vi "Plugin_Validate_Manifest.vi"(8 "error in (no error)":errorcluster={"status"=FALSE, "code"=0, "source"="\"\""}, 10 "target capability":string, 11 "PluginManifest":string) -> (0 "error out":errorcluster={"status"=FALSE, "code"=0, "source"="\"\""}, 2 "status ok":bool, 3 "Allowed/diagnostics":string)   [LabVIEW 2026]
doc: "INTENT: Check plugin interface rights. LOGIC: Check connector signature/version, input/output type, target presence, resource rights and cancellation deadlines."
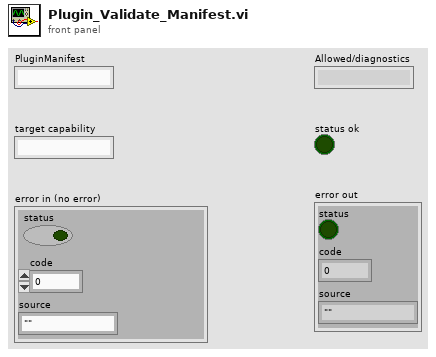
[diagram p1: front panel]
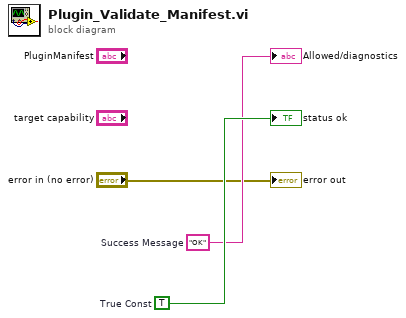
[diagram p0: block diagram]
diagram:
  w3 = TRUE  # True Const
  w2 = "OK"  # Success Message
  "Allowed/diagnostics" <- w2
  "status ok" <- w3
  "error out" <- "error in (no error)"
